vi "test tools list every array has items.vi"(8 "error in (no error)":errorcluster) -> (0 "error out":errorcluster, 3 "body":string)   [LabVIEW 2020, in "MCP Server tests.lvlib"]
doc: "Clients such as ChatGPT/Codex reject the whole tools/list answer when one array schema lacks items. This test walks the complete tools/list answer of the test server, every tool and every nested schema, and counts the objects whose type is array and those of them without items; there must be at least one and none without. The answer is also written to results\\tools-list.json next to this VI, for checking it against other clients' schema rules."
uses:
  MCP Server tests.lvlib
  <vilib>/addons/_JKI Toolkits/Caraya/classes/Test/Test.lvclass
  <vilib>/JDP Science/JSONtext/JSONtext.lvlib
  <vilib>/addons/_JKI Toolkits/Caraya/classes/Assert/Assert.lvclass
panel:
  out "lookup error":errorcluster
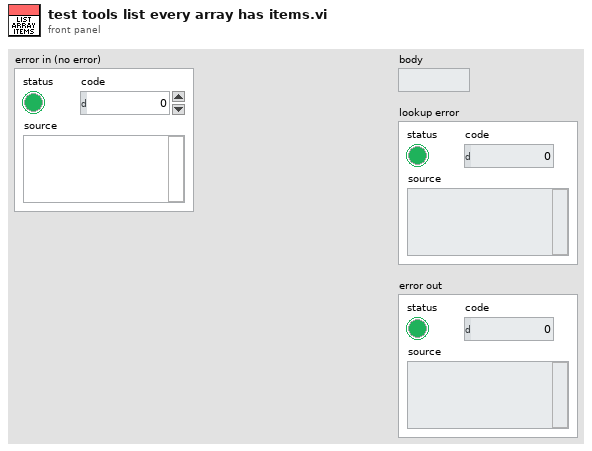
[diagram p1: front panel]
types:
  T1 = typedef "JSONtext.lvlib/JSON Value Type.ctl" = enum16{"Not a JSON Value", "JSON Object", "JSON Array", "String", "Number", "true", "false", "null"}
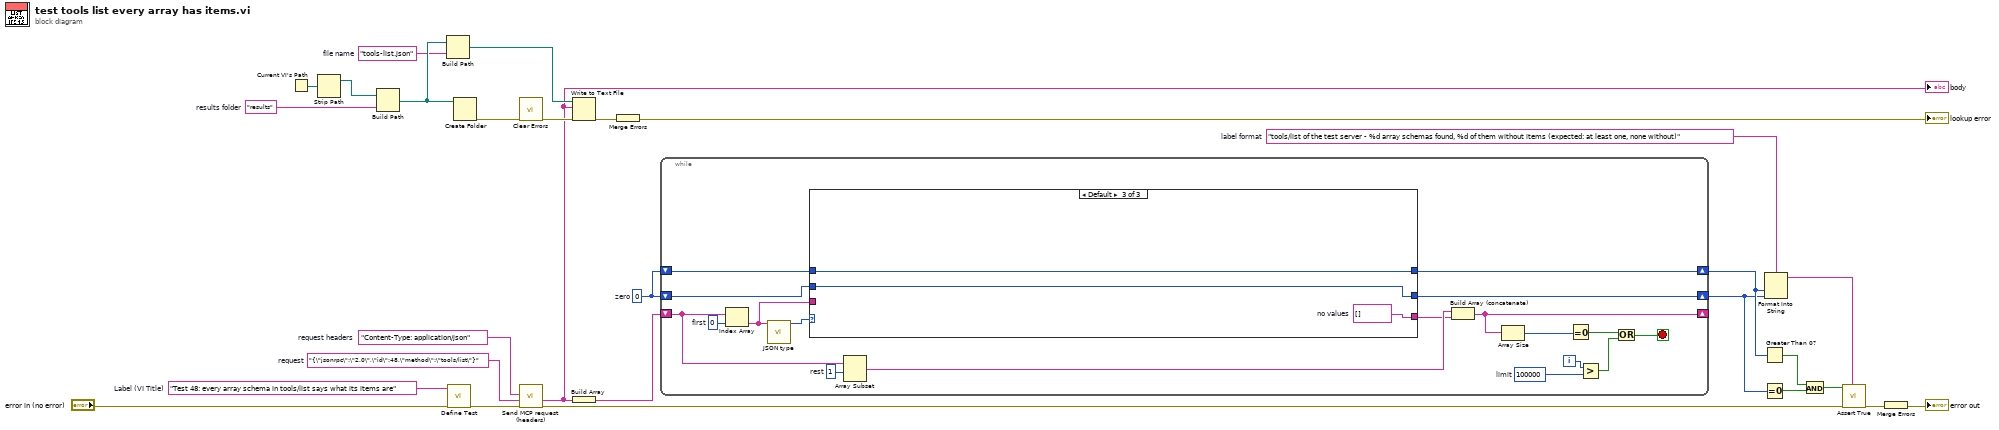
[diagram p0: block diagram]
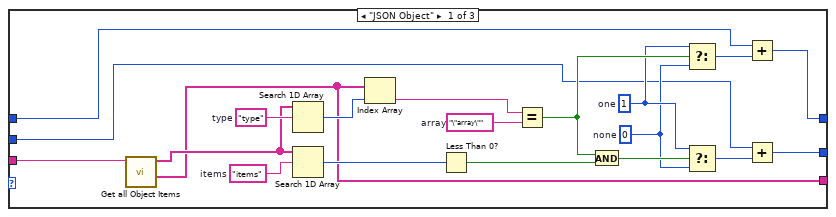
[diagram p2: hidden frame]
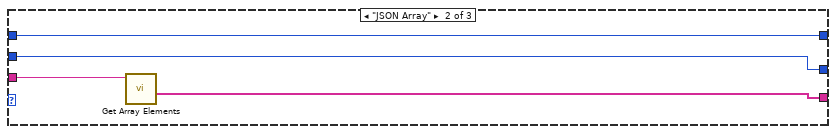
[diagram p3: hidden frame]
diagram:
  w21 = "Content-Type: application/json"  # request headers
  w22 = "tools-list.json"  # file name
  w24 = "results"  # results folder
  w10 = "tools/list of the test server - %d array schemas found, %d of them without items (expected: at least one, none without)"  # label format
  w14 = 0  # zero
  w20 = "{\"jsonrpc\":\"2.0\",\"id\":48,\"method\":\"tools/list\"}"  # request
  w28 = "Test 48: every array schema in tools/list says what its items are"  # Label (VI Title)
  n1 = Current VI's Path() -> (path=w26:path)
  n2 = Strip Path(path=w26) -> (stripped path=w25:path)  [unwired: 1 out]
  n3 = Build Path(base path=w25, name or relative path=w24) -> (appended path=w23:path)
  n4 = Build Path(base path=w23, name or relative path=w22) -> (appended path=w17:path)
  n5 = call <vilib>:"Define Test.vi"("error in (no error)"="error in (no error)", "Label (VI Title)"=w28) -> ("error out"=w19:errorcluster)  [unwired: 8 in, 1 out]
  n6 = Create Folder(path (use dialog)=w23) -> (error out=w18:errorcluster)  [unwired: 2 in, 2 out]
  n7 = call <vilib>:"Clear Errors.vi"("error in (no error)"=w18) -> ("error out"=w16:errorcluster)  [unwired: 5 in, 1 out]
  n8 = call "Send MCP request (headers).vi"("error in (no error)"=w19, "request"=w20, "request headers"=w21) -> ("error out"=w6:errorcluster, "response"=w3:string)  [unwired: 5 in, 2 out]
  "body" <- w3
  n9 = Write to Text File(file (use dialog)=w17, text=w3, error in=w16) -> (error out=w13:errorcluster)  [unwired: 1 in, 2 out]
  n10 = Build Array(w3) -> (w15:string[])
  n11 = Merge Errors(w13) -> (→"lookup error":errorcluster)
  n12 = while {
    shift-right: [w35] -> _
    shift-left: w15 -> [w34]
    shift-right: [w33] -> w12
    shift-left: w14 -> [w32]
    shift-right: [w31] -> w11
    shift-left: w14 -> [w30]
    i -> [w29]
    stop <- w36 stop-if-true
    w46 = 100000  # limit
    w45 = 1  # rest
    w44 = 0  # first
    n13 = Index Array(array=w34, index=w44) -> (element=w43:string)
    n14 = call <vilib>:"JSON type.vi"("JSON"=w43) -> ("JSON Value Type"=w42:T1)  [unwired: 9 in, 1 out]
    n15 = case shown="Default" w42 {
      tunnel: w43 -> [w66 w70 _]
      tunnel: w32 -> [w53 w68 w72]
      tunnel: w30 -> [w51 w67 w71]
      tunnel: [w49 w69 w73] -> w40
      tunnel: [w48 w68 w72] -> w33
      tunnel: [w47 w67 w71] -> w31
      frame "JSON Object" {
        w54 = 0  # none
        w56 = 1  # one
        w59 = "\"array\""  # array
        w63 = "items"  # items
        w65 = "type"  # type
        n16 = call <vilib>:"Get all Object Items.vi"("JSON"=w66) -> ("<JSON>"=w49:string[], "Item Names"=w64:string[])  [unwired: 7 in, 2 out]
        n17 = Search 1D Array(1D array=w64, element=w65) -> (index of element=w62:i32)  [unwired: 1 in]
        n18 = Search 1D Array(1D array=w64, element=w63) -> (index of element=w61:i32)  [unwired: 1 in]
        n19 = Index Array(array=w49, index=w62) -> (element=w60:string)
        n20 = Less Than 0?(x=w61) -> (x < 0?=w58:bool)
        n21 = Equal?(x=w60, y=w59) -> (x = y?=w57:bool)
        n22 = And(x=w57, y=w58) -> (x .and. y?=w55:bool)
        n23 = Select(t=w56, s=w57, f=w54) -> (s? t:f=w52:i32)
        n24 = Select(t=w56, s=w55, f=w54) -> (s? t:f=w50:i32)
        n25 = Add(x=w53, y=w52) -> (x+y=w48:i32)
        n26 = Add(x=w51, y=w50) -> (x+y=w47:i32)
      }
      frame "JSON Array" {
        n27 = call <vilib>:"Get Array Elements.vi"("JSON"=w70) -> ("<JSON>"=w69:string[])  [unwired: 8 in, 2 out]
      }
      frame Default {
        w73 = string[] []  # no values
      }
    }
    n28 = Array Subset(array=w34, index=w45) -> (w41:string[])  [unwired: 1 in]
    n29 = Build Array (concatenate)(w41, w40) -> (w35:string[])
    n30 = Array Size(array=w35) -> (size(s)=w39:i32)
    n31 = Equal To 0?(x=w39) -> (x = 0?=w38:bool)
    n32 = Greater?(x=w29, y=w46) -> (0:w37:bool)
    n33 = Or(x=w38, y=w37) -> (x .or. y?=w36:bool)
  }
  n34 = Greater Than 0?(x=w12) -> (x > 0?=w9:bool)
  n35 = Equal To 0?(x=w11) -> (x = 0?=w8:bool)
  n36 = Format Into String(format string=w10, w12, w11) -> (resulting string=w5:string)  [unwired: 2 in, 1 out]
  n37 = Compound Arithmetic op=AND(w9, w8) -> (w7:bool)
  n38 = call <vilib>:"Assert True.vi"("Label"=w5, "error in (no error)"=w6, "True?"=w7) -> ("error out"=w4:errorcluster)  [unwired: 7 in, 1 out]
  n39 = Merge Errors(w4) -> (→"error out":errorcluster)
